vi "Register.vi"(8 "error in (no error)":errorcluster, 9 "ServerInfo":T1={"DaemonUrl"="http://127.0.0.1:19627/opentool-daemon", "Host"="127.0.0.1", "Port"=8001, "Prefix"="/opentool"}, 10 "StartupFile":path, 11 "ITool.lvclass in":refnum<class "ITool.lvclass">) -> (0 "error out":errorcluster, 1 "DaemonError":string, 2 "Id":string, 3 "ITool.lvclass out":refnum<class "ITool.lvclass">)   [LabVIEW 2017]
uses:
  Server/ITool/ITool.lvclass
  <vilib>/LVH/i3 JSON/JSON Generation/Create Value Files/Create Value - Object.vi
  <vilib>/LVH/i3 JSON/JSON Generation/Add Object Parameter Files/Add Object Parameter - String.vi
  <vilib>/LVH/i3 JSON/JSON Generation/Add Object Parameter Files/Add Object Parameter - Numeric.vi
  <vilib>/LVH/i3 JSON/JSON Generation/Add Object Parameter Files/Add Object Parameter - 1D Array String.vi
  <vilib>/httpClient/POSTBuffer.vi
  <vilib>/LVH/i3 JSON/JSON Parsing/Get Object Parameter Files/Get Object Parameter - String.vi
  <vilib>/LVH/i3 JSON/i3-json.lvlib
  <vilib>/httpClient/LabVIEWHTTPClient.lvlib
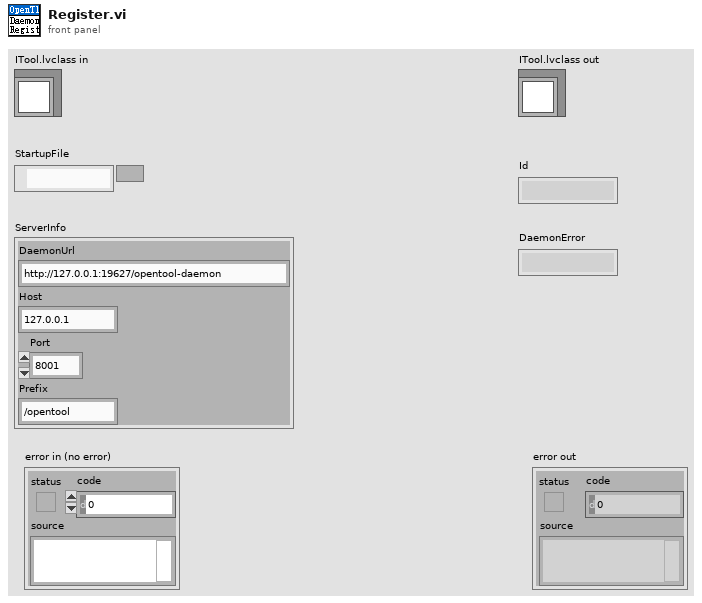
[diagram p1: front panel]
types:
  T1 = cluster{"DaemonUrl":string, "Host":string, "Port":i32, "Prefix":string}
  T2 = typedef "LabVIEWHTTPClient.lvlib/ClientHandle.ctl" = refnum<k1>
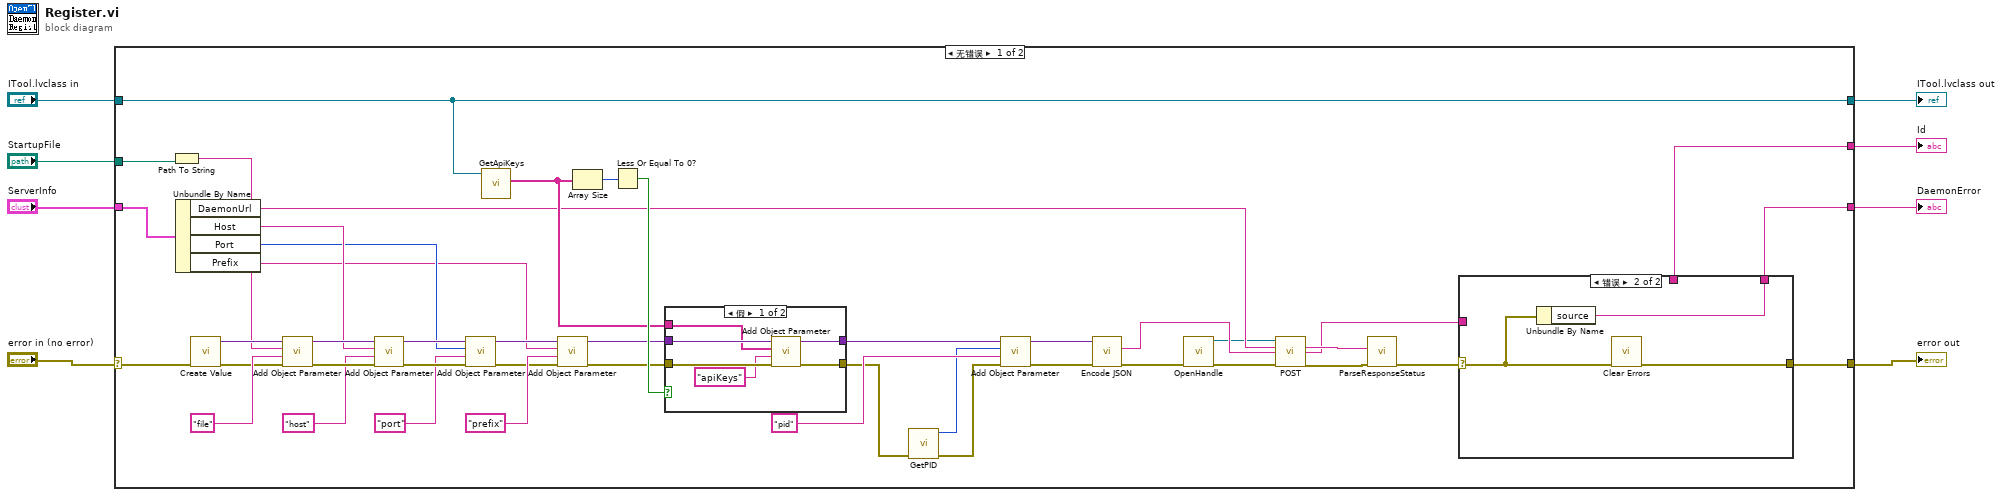
[diagram p0: block diagram]
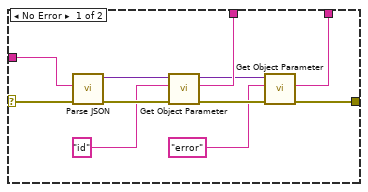
[diagram p2: hidden frame]
diagram:
  n1 = case shown="无错误" "error in (no error)" {
    selector: "error in (no error)" -> [w33 w76]
    tunnel: [w13 w76] -> w7
    tunnel: "ITool.lvclass in" -> [w9 w75]
    tunnel: "StartupFile" -> [w51 _]
    tunnel: "ServerInfo" -> [w31 _]
    tunnel: [w11 _] -> w3
    tunnel: [w10 _] -> w2
    tunnel: [w9 w75] -> w1
    frame No Error {
      n2 = Path To String(path=w51) -> (string=w32:string)
      n3 = Unbundle By Name(w31) -> ("DaemonUrl"=w19:string, "Host"=w30:string, "Port"=w29:i32, "Prefix"=w28:string)
      n4 = call-poly <vilib>:"Create Value.vi"("error in (no error)"=w33) -> ("error out"=w49:errorcluster, "JSON Tree"=w52:variant)  [unwired: 9 in]
      n5 = call-poly <vilib>:"Add Object Parameter.vi"("error in (no error)"=w49, "Name"="file", "String"=w32, "JSON Tree in (JSON Object)"=w52) -> ("error out"=w48:errorcluster, "JSON Tree out (JSON Object)"=w46:variant)  [unwired: 6 in]
      n6 = call-poly <vilib>:"Add Object Parameter.vi"("error in (no error)"=w48, "Name"="host", "String"=w30, "JSON Tree in (JSON Object)"=w46) -> ("error out"=w44:errorcluster, "JSON Tree out (JSON Object)"=w45:variant)  [unwired: 6 in]
      n7 = call-poly <vilib>:"Add Object Parameter.vi"("error in (no error)"=w44, "Name"="port", "Numeric"=w29, "JSON Tree in (JSON Object)"=w45) -> ("error out"=w41:errorcluster, "JSON Tree out (JSON Object)"=w40:variant)  [unwired: 6 in]
      n8 = call "GetApiKeys.vi"("ITool in"=w9) -> ("ApiKeys"=w27:string[])  [unwired: 8 in, 2 out]
      n9 = call-poly <vilib>:"Add Object Parameter.vi"("error in (no error)"=w41, "Name"="prefix", "String"=w28, "JSON Tree in (JSON Object)"=w40) -> ("error out"=w36:errorcluster, "JSON Tree out (JSON Object)"=w37:variant)  [unwired: 6 in]
      n10 = Array Size(array=w27) -> (size(s)=w39:i32)
      n11 = Less Or Equal To 0?(x=w39) -> (x <= 0?=w38:bool)
      n12 = case shown="假" w38 {
        tunnel: w37 -> [w72 w74]
        tunnel: w36 -> [w71 w73]
        tunnel: [w70 w74] -> w35
        tunnel: [w69 w73] -> w26
        tunnel: w27 -> [w68 _]
        frame False {
          n13 = call-poly <vilib>:"Add Object Parameter.vi"("error in (no error)"=w71, "Name"="apiKeys", "1D String"=w68, "JSON Tree in (JSON Object)"=w72) -> ("error out"=w69:errorcluster, "JSON Tree out (JSON Object)"=w70:variant)  [unwired: 6 in]
        }
        frame True {
        }
      }
      n14 = call "GetPID.vi"("error in (no error)"=w26) -> ("error out"=w25:errorcluster, "PID"=w24:i32)  [unwired: 9 in]
      n15 = call-poly <vilib>:"Add Object Parameter.vi"("error in (no error)"=w25, "Name"="pid", "Numeric"=w24, "JSON Tree in (JSON Object)"=w35) -> ("error out"=w22:errorcluster, "JSON Tree out (JSON Object)"=w23:variant)  [unwired: 6 in]
      n16 = call <vilib>:"Encode JSON.vi"("error in (no error)"=w22, "JSON Tree"=w23) -> ("error out"=w21:errorcluster, "String"=w18:string)  [unwired: 4 in]
      n17 = call <vilib>:"OpenHandle.vi"("error in (no error)"=w21) -> ("client handle out"=w17:T2, "error out"=w20:errorcluster)  [unwired: 13 in]
      n18 = call-poly <vilib>:"POST.vi"("client handle"=w17, "url"=w19, "buffer"=w18, "error in (no error)"=w20) -> ("headers"=w15:string, "body"=w12:string, "error out"=w16:errorcluster)  [unwired: 8 in, 1 out]
      n19 = call "ParseResponseStatus.vi"("error in (no error)"=w16, "Headers"=w15) -> ("error out"=w14:errorcluster)  [unwired: 7 in, 2 out]
      n20 = case shown="错误" w14 {
        selector: w14 -> [w63 w65]
        tunnel: [w53 w66] -> w13
        tunnel: w12 -> [w62 _]
        tunnel: [w58 _] -> w11
        tunnel: [w54 w64] -> w10
        frame No Error {
          n21 = call <vilib>:"Parse JSON.vi"("error in (no error)"=w63, "JSON String"=w62) -> ("error out"=w60:errorcluster, "JSON Tree"=w61:variant)  [unwired: 6 in, 2 out]
          n22 = call-poly <vilib>:"Get Object Parameter.vi"("error in (no error)"=w60, "Parameter Name"="id", "JSON Tree In (JSON Object)"=w61) -> ("error out"=w57:errorcluster, "String Value"=w58:string, "JSON Tree Out Passthrough"=w56:variant)  [unwired: 5 in, 1 out]
          n23 = call-poly <vilib>:"Get Object Parameter.vi"("error in (no error)"=w57, "Parameter Name"="error", "JSON Tree In (JSON Object)"=w56) -> ("error out"=w53:errorcluster, "String Value"=w54:string)  [unwired: 5 in, 2 out]
        }
        frame Error {
          n24 = Unbundle By Name(w65) -> ("source"=w64:string)
          n25 = call <vilib>:"Clear Errors.vi"("error in (no error)"=w65) -> ("error out"=w66:errorcluster)  [unwired: 5 in, 1 out]
        }
      }
    }
    frame Error {
    }
  }
  "error out" <- w7
  "Id" <- w3
  "ITool.lvclass out" <- w1
  "DaemonError" <- w2
